vi "Host - Find Path.vi"(6 "Disable Refresh Modules":bool, 7 "Type":enum16{"Slave", "Master"}(ring), 8 "error in (no error)":errorcluster, 9 "Slave Index":u32, 10 "Master Index":u32, 11 "serverName":string="10.0.18.167") -> (0 "error out":errorcluster, 2 "Path":string)   [LabVIEW 2020, in "SEECD System Explorer.lvlib"]
uses:
  SEECD System Explorer.lvlib
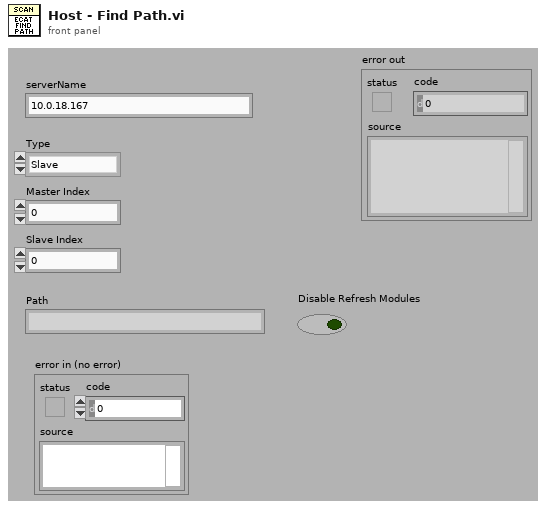
[diagram p1: front panel]
types:
  T1 = typedef "SEECD System Explorer.lvlib/Host - HW Config.ctl" = cluster{"Local Chassis":T2, "Masters":T5[]}
  T2 = typedef "SEECD System Explorer.lvlib/Host - Local Chassis.ctl" = cluster{"Modules":T3[]}
  T3 = typedef "SEECD System Explorer.lvlib/Host - Module.ctl" = cluster{"IOV Ref":string, "Slot":u32, "Model":u32, "All Variables":T4[]}
  T4 = typedef "SEECD System Explorer.lvlib/IOV Container Contents.ctl" = cluster{"Name":string, "Writable":bool, "DataType":variant}
  T5 = typedef "SEECD System Explorer.lvlib/Host - Master.ctl" = cluster{"IOV Ref":string, "Name":string, "Master ID":u32, "Slaves":T6[]}
  T6 = typedef "SEECD System Explorer.lvlib/Host - Slave.ctl" = cluster{"IOV Ref":string, "Name":string, "Position Address":u16, "Bitfile Signature":u8[], "Modules":T3[], "ECAT IOV Contents":T4[]}
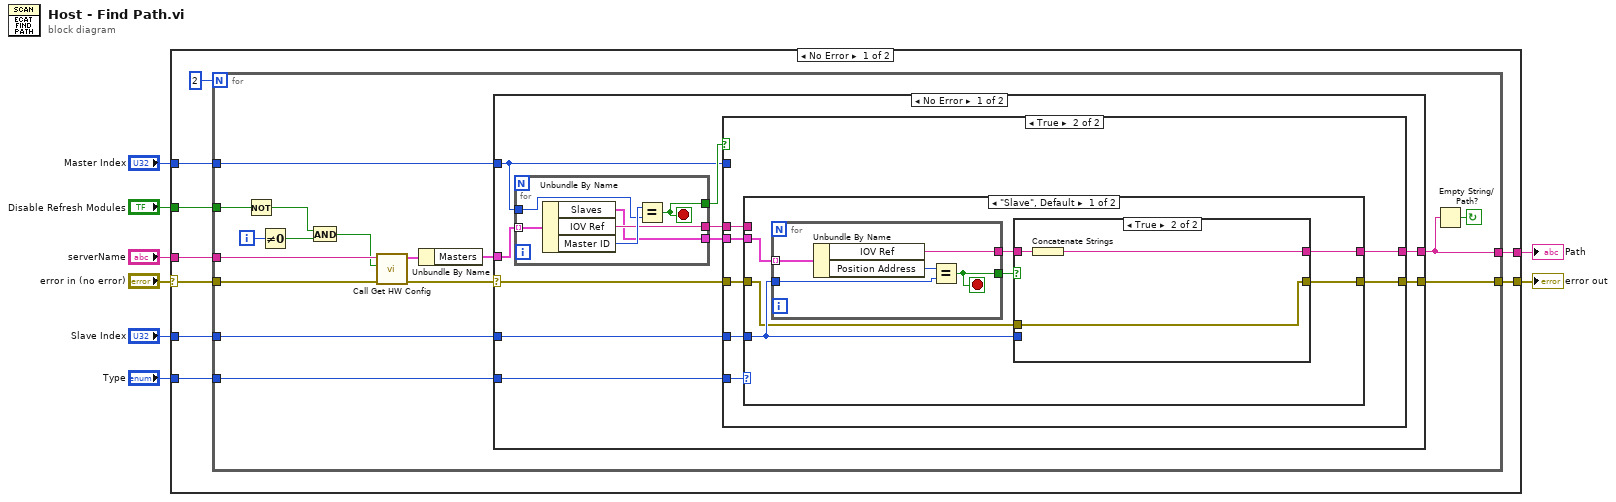
[diagram p0: block diagram]
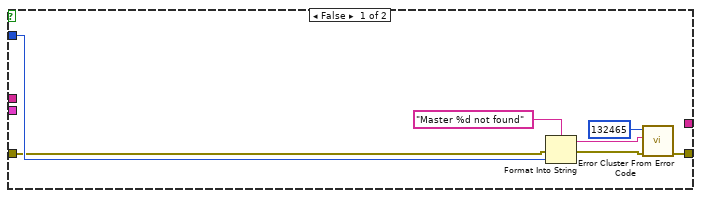
[diagram p2: hidden frame]
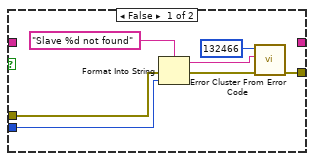
[diagram p3: hidden frame]
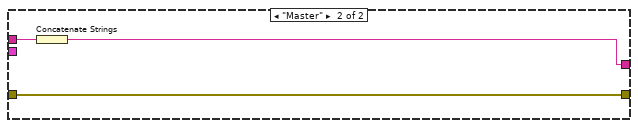
[diagram p4: hidden frame]
diagram:
  n1 = case shown="No Error" "error in (no error)" {
    selector: "error in (no error)" -> [w10 w90]
    tunnel: "Slave Index" -> [w17 _]
    tunnel: "Type" -> [w16 _]
    tunnel: "Master Index" -> [w15 _]
    tunnel: "serverName" -> [w14 _]
    tunnel: [w13 _] -> w4
    tunnel: [w12 w90] -> w3
    tunnel: "Disable Refresh Modules" -> [w9 _]
    frame No Error {
      n2 = for {
        N: 2 -> [_]
        tunnel: w17 -> [w33]
        tunnel: w16 -> [w32]
        tunnel: w15 -> [w31]
        tunnel: w10 -> [w30]
        tunnel: w14 -> [w29]
        tunnel: [w22] -> w13
        tunnel: [w25] -> w12
        tunnel: w9 -> [w19]
        i -> [w24]
        stop <- w23 continue-if-true
        n3 = Not(x=w19) -> (.not. x?=w18:bool)
        n4 = Not Equal To 0?(x=w24) -> (x != 0?=w21:bool)
        n5 = And(x=w18, y=w21) -> (x .and. y?=w20:bool)
        n6 = call "Call Get HW Config.vi"("error in"=w30, "Refresh Modules"=w20, "serverName"=w29) -> ("error out"=w28:errorcluster, "HW Config"=w27:T1)  [unwired: 7 in]
        n7 = Unbundle By Name(w27) -> ("Masters"=w26:T5[])
        n8 = case shown="No Error" w28 {
          selector: w28 -> [w35 w89]
          tunnel: w26 -> [w40 _]
          tunnel: w31 -> [w39 _]
          tunnel: w33 -> [w38 _]
          tunnel: w32 -> [w37 _]
          tunnel: [w36 _] -> w22
          tunnel: [w34 w89] -> w25
          frame No Error {
            n9 = for {
              tunnel: [w88] -> w41
              tunnel: w40 -> [w87] mode=indexing
              tunnel: w39 -> [w85]
              tunnel: [w84] -> w42
              tunnel: [w83] -> w43
              stop <- w88 stop-if-true
              n10 = Unbundle By Name(w87) -> ("Slaves"=w83:T6[], "IOV Ref"=w84:string, "Master ID"=w86:u32)
              n11 = Equal?(x=w86, y=w85) -> (x = y?=w88:bool)
            }
            n12 = case shown="True" w41 {
              tunnel: w42 -> [_ w56]
              tunnel: w37 -> [_ w57]
              tunnel: [_ w55] -> w36
              tunnel: w38 -> [_ w54]
              tunnel: w43 -> [_ w53]
              tunnel: w39 -> [w46 _]
              tunnel: w35 -> [w45 w51]
              tunnel: [w44 w52] -> w34
              frame False {
                n13 = Format Into String(format string="Master %d not found", error in=w45, w46) -> (resulting string=w48:string, error out=w47:errorcluster)  [unwired: 1 in]
                n14 = call <vilib>:"Error Cluster From Error Code.vi"("error in (no error)"=w47, "error message (\"\")"=w48, "error code (0)"=132465) -> ("error out"=w44:errorcluster)  [unwired: 6 in]
              }
              frame True {
                n15 = case shown="\"Slave\", Default" w57 {
                  tunnel: w56 -> [_ w81]
                  tunnel: [w63 w80] -> w55
                  tunnel: w54 -> [w62 _]
                  tunnel: w53 -> [w61 _]
                  tunnel: [w58 w82] -> w52
                  tunnel: w51 -> [w59 w82]
                  frame "Slave", Default {
                    n16 = for {
                      tunnel: w62 -> [w79]
                      tunnel: [w78] -> w64
                      tunnel: w61 -> [w77] mode=indexing
                      tunnel: [w75] -> w60
                      stop <- w78 stop-if-true
                      n17 = Unbundle By Name(w77) -> ("IOV Ref"=w75:string, "Position Address"=w76:u16)
                      n18 = Equal?(x=w76, y=w79) -> (x = y?=w78:bool)
                    }
                    n19 = case shown="True" w64 {
                      tunnel: [_ w72] -> w63
                      tunnel: w62 -> [w67 _]
                      tunnel: w60 -> [_ w73]
                      tunnel: w59 -> [w66 w74]
                      tunnel: [w65 w74] -> w58
                      frame False {
                        n20 = Format Into String(format string="Slave %d not found", error in=w66, w67) -> (resulting string=w69:string, error out=w68:errorcluster)  [unwired: 1 in]
                        n21 = call <vilib>:"Error Cluster From Error Code.vi"("error in (no error)"=w68, "error message (\"\")"=w69, "error code (0)"=132466) -> ("error out"=w65:errorcluster)  [unwired: 6 in]
                      }
                      frame True {
                        n22 = Concatenate Strings(w73) -> (w72:string)
                      }
                    }
                  }
                  frame "Master" {
                    n23 = Concatenate Strings(w81) -> (w80:string)
                  }
                }
              }
            }
          }
          frame Error {
          }
        }
        n24 = Empty String/Path?(string/path=w22) -> (empty?=w23:bool)
      }
    }
    frame Error {
    }
  }
  "error out" <- w3
  "Path" <- w4
